vi "VIH Project Tree - Rename Item.vi"(5 "Set Focus (T)":bool=TRUE, 7 "Ensure visible (T)":bool=TRUE, 8 "error in":errorcluster, 9 "New Item Name":string, 10 "Item Tag":string, 11 "Project Tree":T1) -> (0 "error out":errorcluster, 2 "dup Item Tag":string, 3 "dup Project Tree":T1)   [LabVIEW 2014]
doc: "::: VI Helpeks :::\nCopyright (c) 2000-2026 Konstantin Shifershteyn. All rights reserved."
uses:
  VIH Project Tree Typedef - Tree Refnum.ctl
panel:
  # "VI Helpeks\nCopyright (c) 2012-2026 Konstantin Shifershteyn"
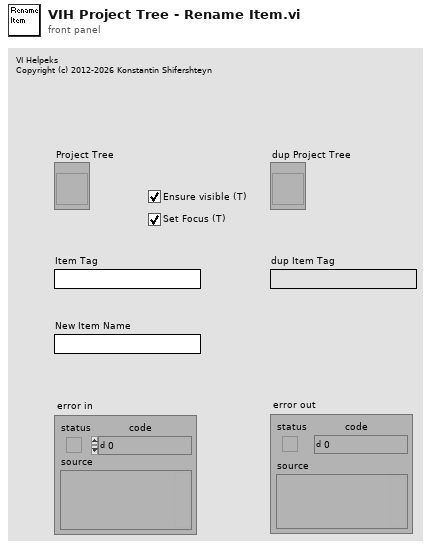
[diagram p1: front panel]
types:
  T1 = typedef "VIH Project Tree Typedef - Tree Refnum.ctl" = refnum<vi>
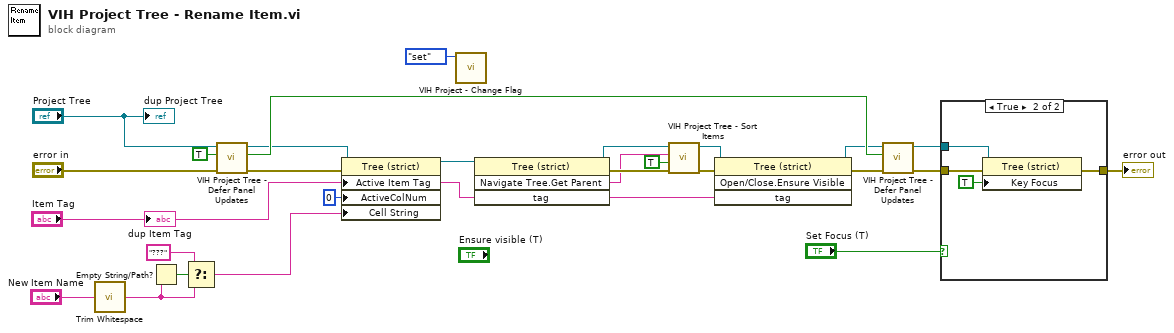
[diagram p0: block diagram]
diagram:
  n1 = call <vilib>:"Trim Whitespace.vi"("string"="New Item Name") -> ("trimmed string"=w19:string)  [unwired: 1 in]
  n2 = Empty String/Path?(string/path=w19) -> (empty?=w18:bool)
  n3 = Select(t="???", s=w18, f=w19) -> (s? t:f=w16:string)
  n4 = call "VIH Project Tree - Defer Panel Updates.vi"("error in"="error in", "Defer Panel Updates (F)"=TRUE, "Project Tree"="Project Tree") -> ("error out"=w22:errorcluster, "Previous Defer status"=w26:bool, "dup Project Tree"=w21:T1)  [unwired: 6 in]
  n5 = property class="Tree (strict)"(reference=w21, error in=w22, "Active Item Tag"="Item Tag", "ActiveColNum"=0 ("Active Cell:Active Column Number"), "Cell String"=w16) -> (reference out=w15:T1)  [unwired: 1 out]
  n6 = call "VIH Project - Change Flag.vi"("cmd (get)"=enum16{"get", "set", "reset"}."set") -> ()  [unwired: 9 in, 2 out]
  n7 = invoke class="Tree (strict)" method="Navigate Tree.Get Parent"(reference=w15, "tag"="Item Tag") -> (reference out=w13:T1, error out=w14:errorcluster, "Navigate Tree:Get Parent"=w11:string)  [unwired: 2 in, 1 out]
  n8 = call "VIH Project Tree - Sort Items.vi"("error in"=w14, "Recursively (T)"=TRUE, "Parent Tag"=w11, "Project Tree"=w13) -> ("error out"=w8:errorcluster, "dup Project Tree"=w7:T1)  [unwired: 5 in, 1 out]
  n9 = invoke class="Tree (strict)" method="Open/Close.Ensure Visible"(reference=w7, error in=w8, "tag"="Item Tag") -> (reference out=w6:T1, error out=w5:errorcluster)  [unwired: 1 in, 2 out]
  n10 = call "VIH Project Tree - Defer Panel Updates.vi"("error in"=w5, "Defer Panel Updates (F)"=w26, "Project Tree"=w6) -> ("error out"=w4:errorcluster, "dup Project Tree"=w3:T1)  [unwired: 6 in, 1 out]
  n11 = case shown="True" "Set Focus (T)" {
    tunnel: w4 -> [w28 w32]
    tunnel: w3 -> [_ w31]
    tunnel: [w28 w30] -> w2
    frame False {
    }
    frame True {
      n12 = property class="Tree (strict)"(reference=w31, error in=w32, "Key Focus"=TRUE) -> (error out=w30:errorcluster)  [unwired: 1 out]
    }
  }
  "error out" <- w2
  "dup Project Tree" <- "Project Tree"
  "dup Item Tag" <- "Item Tag"
